vi "Test Dual Relay.vi"() -> ()   [LabVIEW 2021]
uses:
  USB Relay Control.lvlib
panel:
  in  "index":i32
  out "error out":errorcluster
  in  "On / Off":bool=TRUE
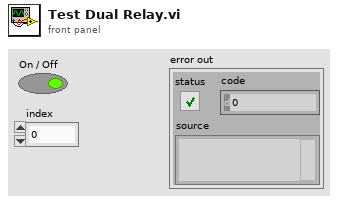
[diagram p1: front panel]
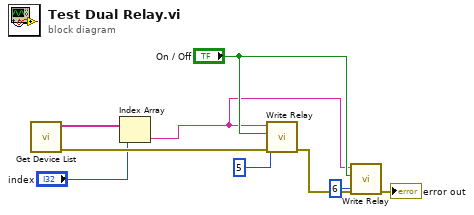
[diagram p0: block diagram]
diagram:
  n1 = call "Get Device List.vi"() -> ("error out"=w3:errorcluster, "Device List"=w5:string[])  [unwired: 10 in]
  n2 = Index Array(array=w5, index="index") -> (element=w4:string)
  n3 = call "Write Relay.vi"("error in (no error)"=w3, "Relay (1 based)"=u8 5, "On / Off"="On / Off", "Device"=w4) -> ("error out"=w7:errorcluster)  [unwired: 7 in]
  n4 = call "Write Relay.vi"("error in (no error)"=w7, "Relay (1 based)"=u8 6, "On / Off"="On / Off", "Device"=w4) -> ("error out"=→"error out":errorcluster)  [unwired: 7 in]
